vi "InitFromXML.vi"(8 "error in (no error)":errorcluster, 10 "XML":string, 11 "New in":refnum<class "New.lvclass">) -> (0 "error out":errorcluster, 3 "New out":refnum<class "New.lvclass">)   [LabVIEW 2023, in "GettingStartedWindow.lvlib" / "New.lvclass"]
uses:
  <resource>/modes/FRC/Classes/New/New.lvclass
  <resource>/modes/FRC/Classes/New/NewDocType.ctl
  <resource>/modes/FRC/Classes/New/New.lvclass/New.ctl
  <resource>/modes/FRC/Classes/ClickableText/ClickableText.lvclass
  <resource>/modes/FRC/GettingStartedWindow.lvlib
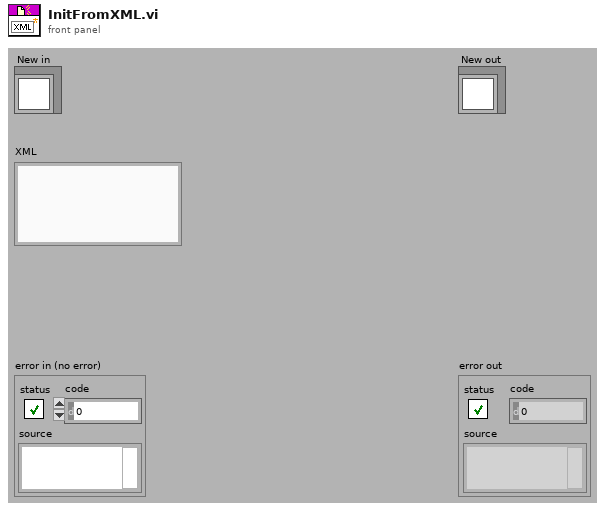
[diagram p1: front panel]
types:
  T1 = typedef "GettingStartedWindow.lvlib/New.lvclass/NewDocType.ctl" = enum16{"dialog", "VI", "project"}
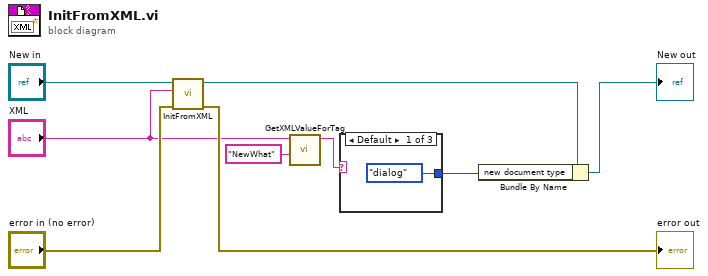
[diagram p0: block diagram]
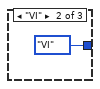
[diagram p2: hidden frame]
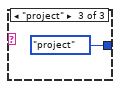
[diagram p3: hidden frame]
diagram:
  n1 = call-parent "InitFromXML.vi"("error in (no error)"="error in (no error)", "XML"="XML", "ClickableText in"="New in") -> ("error out"=→"error out":errorcluster, "ClickableText out"=w4:refnum<class "New.lvclass">)  [unwired: 7 in]
  n2 = call <resource>:"GetXMLValueForTag.vi"("tag"="NewWhat", "XML"="XML") -> ("value"=w3:string)  [unwired: 8 in, 1 out]
  n3 = case shown="Default" w3 {
    tunnel: [NewDocType."dialog" ("new document type") NewDocType."VI" ("new document type") NewDocType."project" ("new document type")] -> w1
    frame Default {
    }
    frame "VI" {
    }
    frame "project" {
    }
  }
  n4 = Bundle By Name(cluster=w4, "new document type"=w1) -> (→"New out":refnum<class "New.lvclass">)
